vi "Append to string.vi"(8 "byte limit":i32=10000, 9 "string":string, 11 "Str Refnum":refnum<vi>) -> ()   [LabVIEW 2023]
doc: "Append string and as a new line. Periodically crop history to size bytes (10k default)."
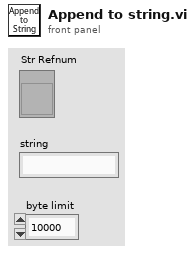
[diagram p1: front panel]
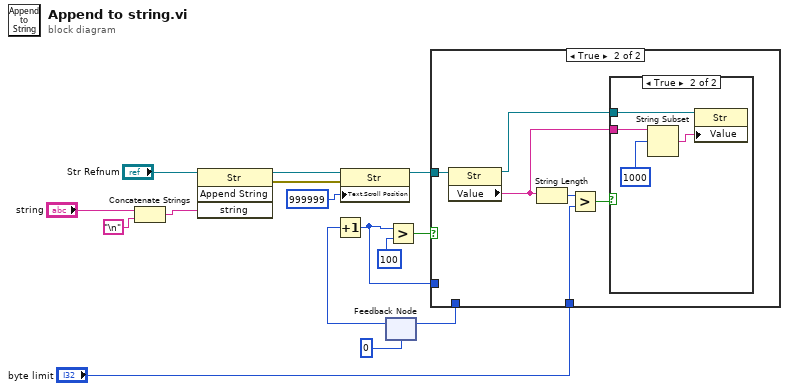
[diagram p0: block diagram]
diagram:
  n1 = Concatenate Strings("string", "\n") -> (w14:string)
  n2 = invoke on="Invoke Node" class="Str" method="Append String"(reference="Str Refnum", "string"=w14) -> (reference out=w11:refnum<vi>, error out=w13:errorcluster)  [unwired: 2 in, 2 out]
  n3 = property on="Property Node" class="Str"(reference=w11, error in=w13, "Text.Scroll Position"=u32 999999) -> (reference out=w3:refnum<vi>)  [unwired: 1 out]
  n4 = feedback #1(0) -> (w10:i32)
  n5 = Increment(x=w10) -> (x+1=w6:i32)
  n6 = Greater?(x=w6, y=100) -> (0:w8:bool)
  n7 = case shown="True" w8 {
    tunnel: w6 -> [w16 _]
    tunnel: [w16 _] -> w5
    tunnel: w3 -> [_ w19]
    tunnel: "byte limit" -> [_ w17]
    frame False {
    }
    frame True {
      # "when over 10k"
      n8 = property on="Property Node" class="Str"(reference=w19) -> (reference out=w18:refnum<vi>, "Value"=w20:string)  [unwired: 1 in, 1 out]
      n9 = String Length(string=w20) -> (length=w22:i32)
      n10 = Greater?(x=w22, y=w17) -> (0:w21:bool)
      n11 = case shown="True" w21 {
        tunnel: w20 -> [_ w26]
        tunnel: w18 -> [_ w23]
        frame False {
        }
        frame True {
          # "shrink by 1k"
          n12 = String Subset(string=w26, offset (0)=1000) -> (substring=w24:string)  [unwired: 1 in]
          n13 = property on="Property Node" class="Str"(reference=w23, "Value"=w24) -> ()  [unwired: 1 in, 2 out]
        }
      }
    }
  }
  n14 = feedback-in #1(w5) -> ()
